vi "PD23X Test.vi"() -> ()   [LabVIEW 2019]
uses:
  <instrlib>/_KELLER RS485 Library/Public/Type Definitions/Information.ctl
  <instrlib>/_KELLER RS485 Library/Public/Type Definitions/Status byte.ctl
  <instrlib>/_KELLER RS485 Library/Public/Type Definitions/Baud Rate.ctl
  <vilib>/Platform/TimedLoop/XDataNode/timing_clust.ctl
  <vilib>/Platform/TimedLoop/XDataNode/nitl_modes.ctl
  <vilib>/Platform/TimedLoop/XDataNode/wakeup.ctl
  <instrlib>/_KELLER RS485 Library/Public/Type Definitions/Channel.ctl
  <vilib>/platform/TimedLoop/XDataNode/XDataNode.xnode
  <instrlib>/_KELLER RS485 Library/KELLER RS485 Library.lvlib
  <vilib>/Platform/TimedLoop/XDataNode/XDNodeRunTimeDep.lvlib
  <vilib>/Analysis/NI_AALBase.lvlib
panel:
  out "Finished Late? [i-1]":bool
  in  "Address":u8=1
  out "time (ms)":u32
  out "stdev":dbl format="%0.6f"
  out "mean":dbl format="%0.6f"
  out "Array":sgl[](array[numeric])
  in  "Amount":i32
  in  "Period":i64=35
  out "error out":errorcluster
  out "Serial number out":u32
  out "Status":T1
  out "Firmware Version out":string
  out "Information out":T2
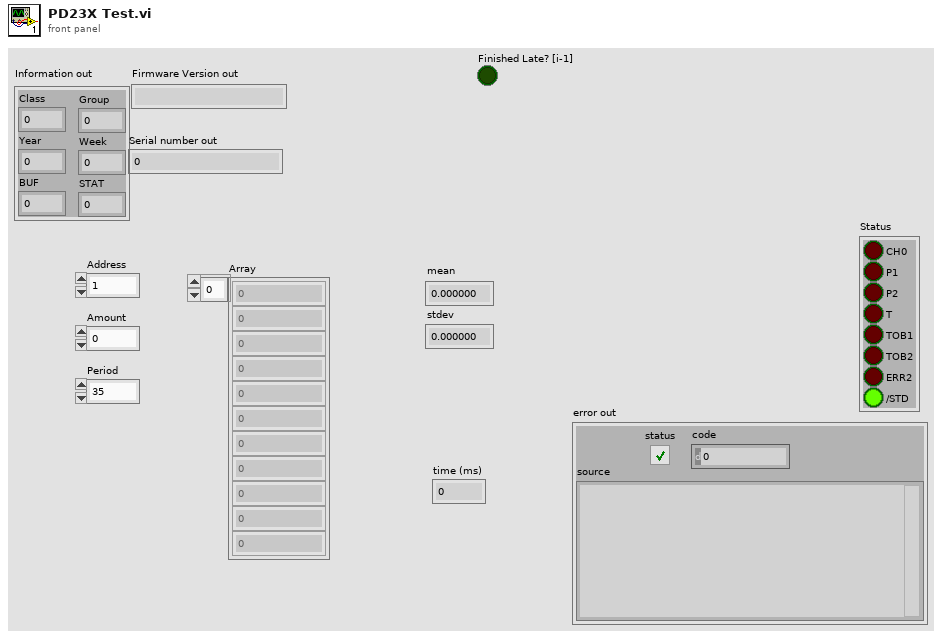
[diagram p1: front panel]
types:
  T1 = typedef "KELLER RS485 Library.lvlib/Status byte.ctl" = cluster{"CH0":bool, "P1":bool, "P2":bool, "T":bool, "TOB1":bool, "TOB2":bool, "ERR2":bool, "/STD":bool}
  T2 = typedef "KELLER RS485 Library.lvlib/Information.ctl" = cluster{"Class":u8, "Group":u8, "Year":u8, "Week":u8, "BUF":u8, "STAT":u8}
  T3 = typedef "KELLER RS485 Library.lvlib/Baud Rate.ctl" = enum16{"9600bd", "115200bd"}
  T4 = typedef "KELLER RS485 Library.lvlib/Bus.ctl" = cluster{"VISA":refnum<visa-resource-name>, "Baud Rate ":T3, "Timeout":u32, "Echo?":bool, "Wait before transmit":u32}
  T5 = typedef "XDNodeRunTimeDep.lvlib/timing_clust.ctl" = cluster{"Expected End [f-1]":u64, "Actual End [f-1]":u64, "Finished Late? [f-1]":bool, "Expected End [i-1]":u64, "Actual End [i-1]":u64, "Finished Late? [i-1]":bool, "Expected Start [i]":u64, "Actual Start [i]":u64, "Expected Start [f]":u64, "Actual Start [f]":u64, "Source Name":string, "Structure Name":string, "Period":i64, "Deadline":i64, "Offset":i64, "Start":i64, "Priority":i32, "Timeout":i32, "Mode":T6, "Wakeup Reason":T7, "Error":errorcluster, "Source Type":string, "Secondary Source Type":string, "Global End Time":u64, "Global Start Time":u64, "Frame Duration":u64, "Iteration Duration":u64, "Assigned CPU":i32, "I/O Scan Engine Mode":u32}
  T6 = typedef "XDNodeRunTimeDep.lvlib/nitl_modes.ctl" = enum32{"No Change", "Process missed periods, maintain original phase", "Discard missed periods, maintain original phase", "Process missed periods, ignore original phase", "Discard missed periods, ignore original phase"}
  T7 = typedef "XDNodeRunTimeDep.lvlib/wakeup.ctl" = enum32{"Normal", "Aborted", "Asynchronous wakeup", "Timing source error", "Timed loop error", "Timeout"}
  T8 = typedef "KELLER RS485 Library.lvlib/Channel.ctl" = enum16{"CH0", "P1", "P2", "T", "TOB1", "TOB2", "TE", "CH7", "CH8", "CH9", "ConTc", "ConRaw", "CH12"}
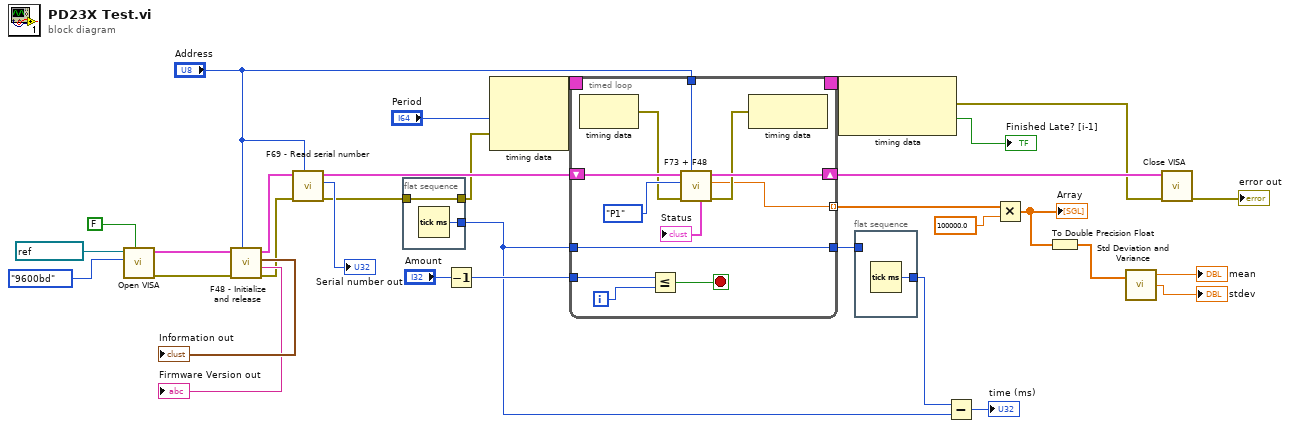
[diagram p0: block diagram]
diagram:
  n1 = call <instrlib>:"Open VISA.vi"("Echo? (T)"=FALSE, "Baud Rate (9600bd)"=Baud_Rate."9600bd", "VISA resource name"=refnum<visa-resource-name> "COM11") -> ("error out"=w30:errorcluster, "Bus out"=w31:T4)  [unwired: 7 in]
  n2 = call <instrlib>:"F48 - Initialize and release.vi"("Address (250)"="Address", "error in (no error)"=w30, "Bus in"=w31) -> ("error out"=w26:errorcluster, "Firmware Version out"=→"Firmware Version out":string, "Information out"=→"Information out":T2, "Bus out"=w27:T4)  [unwired: 5 in]
  n3 = call <instrlib>:"F69 - Read serial number.vi"("Address (250)"="Address", "error in (no error)"=w26, "Bus in"=w27) -> ("error out"=w11:errorcluster, "Serial number out"=→"Serial number out":u32, "Bus out"=w21:T4)  [unwired: 6 in]
  n4 = flat-sequence {
    tunnel: [w35] -> w8
    tunnel: w11 -> [w34]
    tunnel: [w34] -> w10
    frame #0 {
      n5 = Tick Count (ms)() -> (millisecond timer value=w35:u32)
    }
  }
  n6 = Decrement(x="Amount") -> (x-1=w12:i32)
  n7 = node-c288("Period", w10) -> (w23:T5)  [unwired: 1 in]
  n8 = timed-loop {
    timing: w23 -> [_]
    timing-out: [_] -> w22
    shift-right: [w46] -> w18
    shift-left: w21 -> [w47]
    tunnel: w12 -> [w44]
    tunnel: w8 -> [w38]
    tunnel: [w38] -> w15
    tunnel: [w37] -> w5 mode=indexing
    tunnel: "Address" -> [w36]
    i -> [w43]
    stop <- w42 stop-if-true
    n9 = node-c288() -> (w41:errorcluster)  [unwired: 1 in]
    n10 = Less Or Equal?(x=w44, y=w43) -> (x <= y?=w42:bool)
    n11 = call <instrlib>:"F73 + F48.vi"("Address (250)"=w36, "error in (no error)"=w41, "Channel (P1)"=Channel."P1", "Bus in"=w47) -> ("error out"=w40:errorcluster, "Value as Single"=w37:sgl, "Bus out"=w46:T4, "Status (STAT)"=→"Status":T1)  [unwired: 3 in, 1 out]
    n12 = node-c288(w40) -> ()  [unwired: 1 out]
  }
  n13 = node-c288(w22) -> (w17:errorcluster, →"Finished Late? [i-1]":bool)
  n14 = flat-sequence {
    tunnel: w15 -> [_]
    tunnel: [w53] -> w14
    frame #0 {
      n15 = Tick Count (ms)() -> (millisecond timer value=w53:u32)
    }
  }
  n16 = Subtract(x=w14, y=w8) -> (x-y=→"time (ms)":u32)
  n17 = Multiply(x=w5, y=sgl 100000.0) -> (x*y=w1:sgl[])
  "Array" <- w1
  n18 = To Double Precision Float(number=w1) -> (double precision float=w4:dbl[])
  n19 = call <vilib>:"Std Deviation and Variance.vi"("X"=w4) -> ("mean"=→"mean":dbl, "standard deviation"=→"stdev":dbl)  [unwired: 1 in, 1 out]
  n20 = call <instrlib>:"Close VISA.vi"("error in (no error)"=w17, "Bus in"=w18) -> ("error out"=→"error out":errorcluster)  [unwired: 9 in]
